vi "VM wrappers - Error Handler.vi"(6 "extra msg":string, 7 "VC Handle":T2=-1, 8 "error before":errorcluster, 9 "VarMan error":T1 items=["No error", "Invalid variable type", "Variable not found", "Variable already exists", "Invalid context handle", "Input error", "Invalid data format", "No history attached", "History already attached", "Invalid history parameters", "Wrong variable name", "Wrong alias name", "Non-unique alias", "Alias not found", "No alias associated", "Alias already associated", "Wrong context name", "Non-unique context name", "Context name not found", "Invalid parameter", "Generic error", "Memory Full", "Unrecognized LV error", "Unknown error code"], 10 "show name spec (F)":bool, 11 "name spec":string) -> (0 "error out":errorcluster, 1 "dup VarMan error":T1 items=["No error", "Invalid variable type", "Variable not found", "Variable already exists", "Invalid context handle", "Input error", "Invalid data format", "No history attached", "History already attached", "Invalid history parameters", "Wrong variable name", "Wrong alias name", "Non-unique alias", "Alias not found", "No alias associated", "Alias already associated", "Wrong context name", "Non-unique context name", "Context name not found", "Invalid parameter", "Generic error", "Memory Full", "Unrecognized LV error", "Unknown error code"])   [LabVIEW 2021]
doc: "::: CalcExpress Toolkit :::\nCopyright (c) 2000-2026 Konstantin Shifershteyn. All rights reserved."
uses:
  cetypes.llb/VarMan Error Code.ctl
  cetypes.llb/VarMan Variable Context Handle.ctl
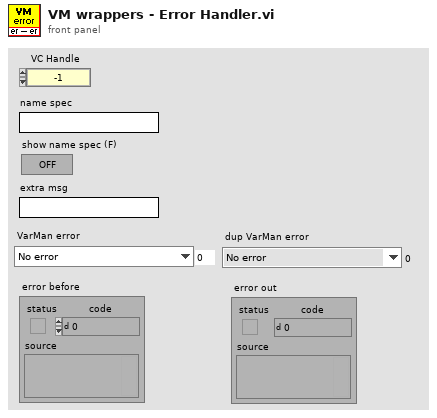
[diagram p1: front panel]
types:
  T1 = typedef "VarMan Error Code.ctl" = u16
  T2 = typedef "VarMan Variable Context Handle.ctl" = i32
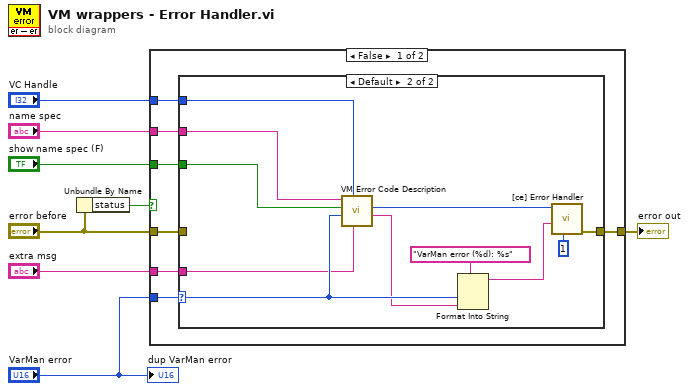
[diagram p0: block diagram]
diagram:
  n1 = Unbundle By Name("error before") -> ("status"=w7:bool)
  n2 = case shown="False" w7 {
    tunnel: [w15 w28] -> w8
    tunnel: "error before" -> [w14 w28]
    tunnel: "VarMan error" -> [w13 _]
    tunnel: "VC Handle" -> [w12 _]
    tunnel: "name spec" -> [w11 _]
    tunnel: "show name spec (F)" -> [w10 _]
    tunnel: "extra msg" -> [w9 _]
    frame False {
      n3 = case shown="Default" w13 {
        selector: w13 -> [_ w26]
        tunnel: [w16 w24] -> w15
        tunnel: w14 -> [w16 _]
        tunnel: w12 -> [_ w20]
        tunnel: w11 -> [_ w19]
        tunnel: w10 -> [_ w18]
        tunnel: w9 -> [_ w17]
        frame 0 {
        }
        frame Default {
          n4 = call "VM Error Code Description.vi"("extra msg"=w17, "VC Handle"=w20, "VarMan Engine error"=w26, "show name spec (F)"=w18, "name spec"=w19) -> ("error description"=w25:string, "VM VI error code"=w23:i32)  [unwired: 4 in, 1 out]
          n5 = Format Into String(format string="VarMan error (%d): %s" ("source"), w26, w25) -> (resulting string=w22:string)  [unwired: 2 in, 1 out]
          n6 = call "[ce] Error Handler.vi"("nesting level"=1, "error reason"=w22, "error code"=w23) -> ("error out"=w24:errorcluster)  [unwired: 7 in, 1 out]
        }
      }
    }
    frame True {
    }
  }
  "error out" <- w8
  "dup VarMan error" <- "VarMan error"
